vi "Initiate TS.vi"(8 "error in":errorcluster, 11 "Water Tunnel Test Stand in":refnum<class "Water Tunnel Test Stand.lvclass">) -> (0 "error out":errorcluster, 3 "Water Tunnel Test Stand out":refnum<class "Water Tunnel Test Stand.lvclass">)   [LabVIEW 2019, in "Test Stands.lvlib" / "Water Tunnel Test Stand.lvclass"]
uses:
  Water Tunnel Test Stand.lvclass
  Results/Results Method.ctl
  Results/Water Tunnel Results/Water Tunnel Results.lvclass
  Generic Test Stand/TS Panel Method.ctl
  Results/Results.lvlib
  Generic Test Stand/Generic Test Stand.lvclass
  DAC/Water Tunnel/Traverse/DAC Traverse.lvclass
  C:/Users/wg/Documents/LV_Projects/test-stand/App/DAC/DAC.lvclass
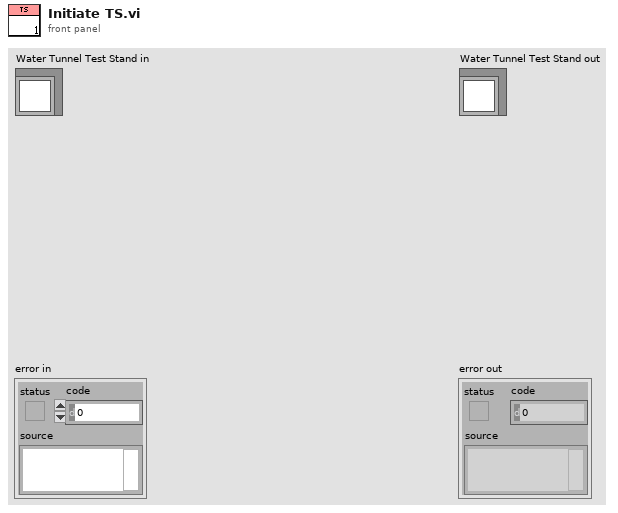
[diagram p1: front panel]
types:
  T1 = typedef "Generic Test Stand.lvclass/TS Panel Method.ctl" = enum16{"Send to Panel", "Receive from Panel"}
  T2 = typedef "Results.lvlib/Results Method.ctl" = enum16{"Get", "Set"}
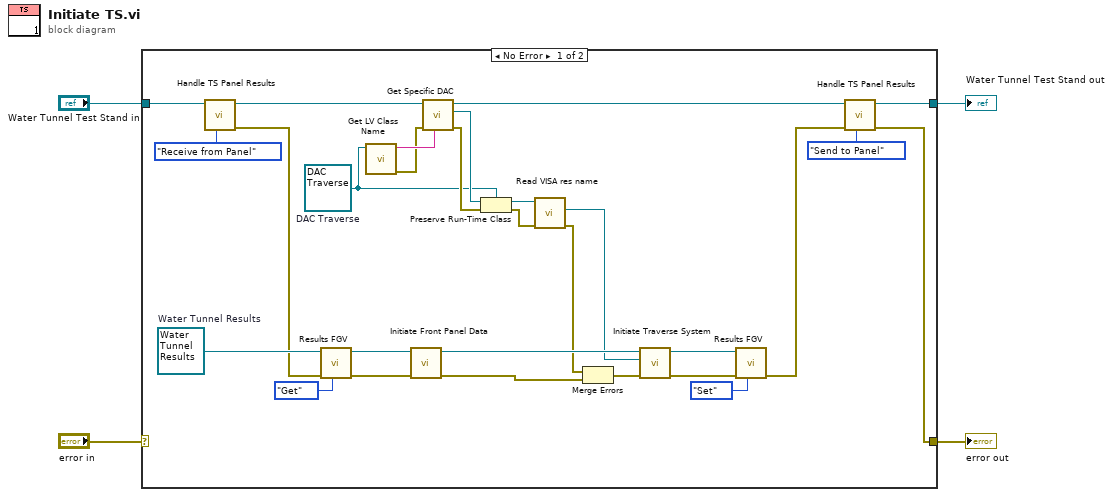
[diagram p0: block diagram]
diagram:
  n1 = case shown="No Error" "error in" {
    selector: "error in" -> [_ w34]
    tunnel: [w21 w34] -> w4
    tunnel: [w24 w33] -> w3
    tunnel: "Water Tunnel Test Stand in" -> [w25 w33]
    frame No Error {
      w12 = refnum<class "DAC Traverse.lvclass"> refnum  # DAC Traverse
      w30 = refnum<class "Water Tunnel Results.lvclass"> refnum  # Water Tunnel Results
      n2 = call-dynamic "Handle TS Panel Results.vi"("Method"=TS_Panel_Method."Receive from Panel", "Water Tunnel Test Stand in"=w25) -> ("error out"=w23:errorcluster, "Water Tunnel Test Stand out"=w17:refnum<class "Water Tunnel Test Stand.lvclass">)  [unwired: 8 in]
      n3 = call-dynamic "Results FGV.vi"("Method"=Results_Method."Get", "error in"=w23, "Water Tunnel Results in"=w30) -> ("error out"=w28:errorcluster, "Water Tunnel  Results out"=w29:refnum<class "Water Tunnel Results.lvclass">)  [unwired: 7 in]
      n4 = call <vilib>:"Get LV Class Name.vi"("object"=w12) -> ("error out"=w15:errorcluster, "class name"=w16:string)  [unwired: 9 in]
      n5 = call "Initiate Front Panel Data.vi"("error in"=w28, "Water Tunnel Results in"=w29) -> ("error out"=w6:errorcluster, "Water Tunnel Results out"=w20:refnum<class "Water Tunnel Results.lvclass">)  [unwired: 8 in]
      n6 = call-dynamic "Get Specific DAC.vi"("DAC Class Name"=w16, "error in"=w15, "Generic Test Stand in"=w17) -> ("error out"=w13:errorcluster, "DAC"=w14:refnum<class "DAC.lvclass">, "Generic Test Stand out"=w9:refnum<class "Water Tunnel Test Stand.lvclass">)  [unwired: 6 in]
      n7 = Preserve Run-Time Class(object in=w14, error in=w13, 2:w12) -> (object out=w11:refnum<class "DAC Traverse.lvclass">, error out=w10:errorcluster)
      n8 = call "Read VISA res name.vi"("error in (no error)"=w10, "DAC Traverse in"=w11) -> ("error out"=w5:errorcluster, "VISA res name"=w8:refnum<visa-resource-name>)  [unwired: 7 in, 1 out]
      n9 = Merge Errors(w5, w6) -> (w7:errorcluster)
      n10 = call "Initiate Traverse System.vi"("error in"=w7, "VISA resource name"=w8, "Water Tunnel Results in"=w20) -> ("error out"=w18:errorcluster, "Water Tunnel Results out"=w19:refnum<class "Water Tunnel Results.lvclass">)  [unwired: 6 in, 1 out]
      n11 = call-dynamic "Results FGV.vi"("Method"=Results_Method."Set", "error in"=w18, "Water Tunnel Results in"=w19) -> ("error out"=w22:errorcluster)  [unwired: 7 in, 1 out]
      n12 = call-dynamic "Handle TS Panel Results.vi"("Method"=TS_Panel_Method."Send to Panel", "error in"=w22, "Water Tunnel Test Stand in"=w9) -> ("error out"=w21:errorcluster, "Water Tunnel Test Stand out"=w24:refnum<class "Water Tunnel Test Stand.lvclass">)  [unwired: 7 in]
    }
    frame Error {
    }
  }
  "error out" <- w4
  "Water Tunnel Test Stand out" <- w3
